vi "截取字符串.vi"(0 "T 1":T2, 1 "标刻内容 2":T1, 5 "T 2":T2, 9 "T 3":T2, 11 "T 4":T2, 12 "T 5":T2, 13 "T 6":T2) -> (4 "标刻内容":T1)   [LabVIEW 2021]
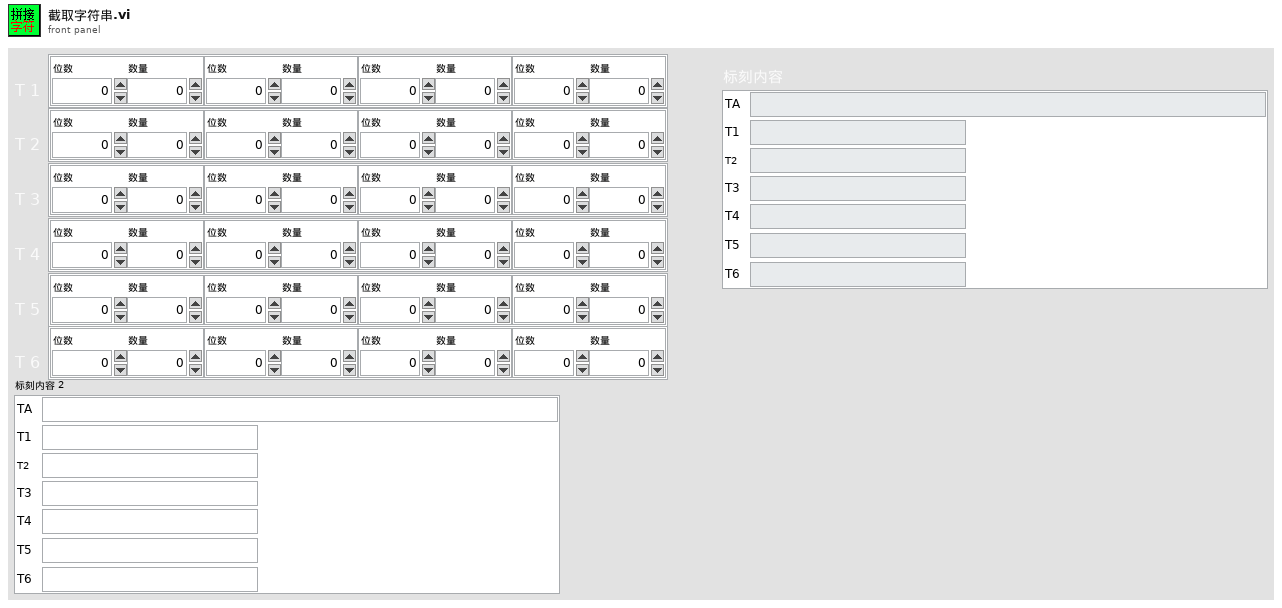
[diagram p1: front panel]
types:
  T1 = typedef "标刻内容.ctl" = cluster{"T1":string, "T2":string, "T3":string, "T4":string, "TA":string, "T5":string, "T6":string}
  T2 = typedef "T码提取设置.ctl" = cluster{"T1 1":cluster{"位数":dbl, "数量":dbl}, "T1 2":cluster{"位数":dbl, "数量":dbl}, "T1 3":cluster{"位数":dbl, "数量":dbl}, "T1 4":cluster{"位数":dbl, "数量":dbl}}
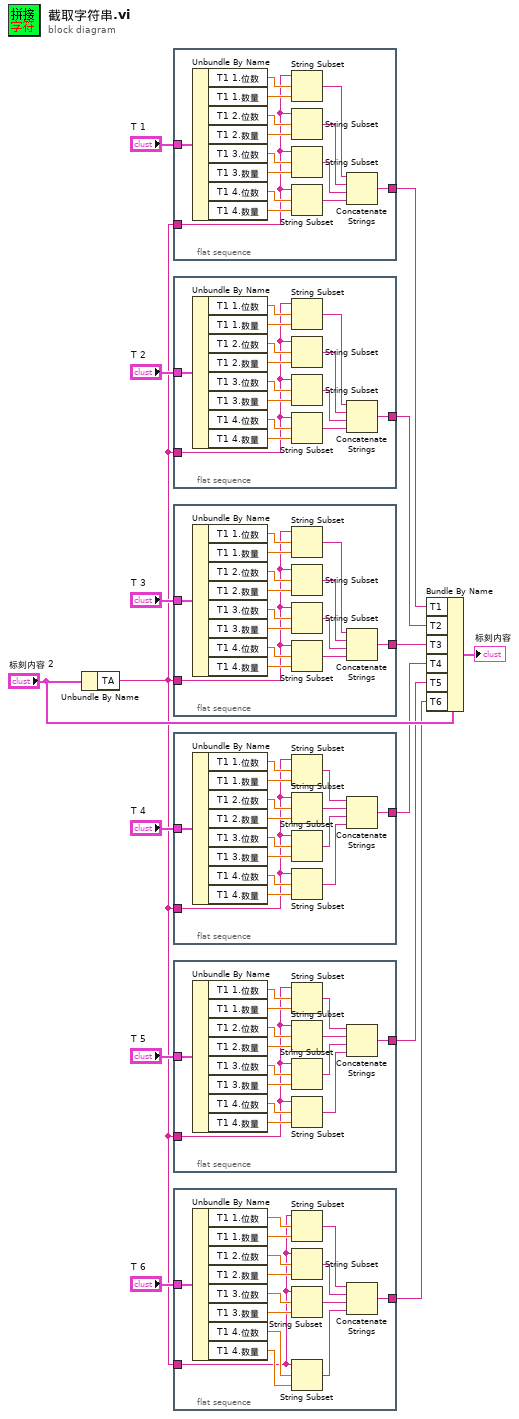
[diagram p0: block diagram]
diagram:
  n1 = Unbundle By Name("标刻内容 2") -> ("TA"=w6:string)
  n2 = flat-sequence {
    tunnel: "T 1" -> [w30]
    tunnel: w6 -> [w21]
    tunnel: [w16] -> w12
    frame #0 {
      n3 = Unbundle By Name(w30) -> ("T1 1.位数"=w29:dbl, "T1 1.数量"=w28:dbl, "T1 2.位数"=w27:dbl, "T1 2.数量"=w26:dbl, "T1 3.位数"=w25:dbl, "T1 3.数量"=w24:dbl, "T1 4.位数"=w23:dbl, "T1 4.数量"=w22:dbl)
      n4 = String Subset(string=w21, offset (0)=w29, length (rest)=w28) -> (substring=w20:string)
      n5 = String Subset(string=w21, offset (0)=w27, length (rest)=w26) -> (substring=w19:string)
      n6 = String Subset(string=w21, offset (0)=w25, length (rest)=w24) -> (substring=w18:string)
      n7 = String Subset(string=w21, offset (0)=w23, length (rest)=w22) -> (substring=w17:string)
      n8 = Concatenate Strings(w20, w19, w18, w17) -> (w16:string)
    }
  }
  n9 = flat-sequence {
    tunnel: "T 2" -> [w45]
    tunnel: [w32] -> w5
    tunnel: w6 -> [w31]
    frame #0 {
      n10 = Unbundle By Name(w45) -> ("T1 1.位数"=w44:dbl, "T1 1.数量"=w43:dbl, "T1 2.位数"=w42:dbl, "T1 2.数量"=w41:dbl, "T1 3.位数"=w40:dbl, "T1 3.数量"=w39:dbl, "T1 4.位数"=w38:dbl, "T1 4.数量"=w37:dbl)
      n11 = String Subset(string=w31, offset (0)=w44, length (rest)=w43) -> (substring=w36:string)
      n12 = String Subset(string=w31, offset (0)=w42, length (rest)=w41) -> (substring=w35:string)
      n13 = String Subset(string=w31, offset (0)=w40, length (rest)=w39) -> (substring=w34:string)
      n14 = String Subset(string=w31, offset (0)=w38, length (rest)=w37) -> (substring=w33:string)
      n15 = Concatenate Strings(w36, w35, w34, w33) -> (w32:string)
    }
  }
  n16 = flat-sequence {
    tunnel: "T 3" -> [w60]
    tunnel: w6 -> [w51]
    tunnel: [w46] -> w4
    frame #0 {
      n17 = Unbundle By Name(w60) -> ("T1 1.位数"=w59:dbl, "T1 1.数量"=w58:dbl, "T1 2.位数"=w57:dbl, "T1 2.数量"=w56:dbl, "T1 3.位数"=w55:dbl, "T1 3.数量"=w54:dbl, "T1 4.位数"=w53:dbl, "T1 4.数量"=w52:dbl)
      n18 = String Subset(string=w51, offset (0)=w59, length (rest)=w58) -> (substring=w50:string)
      n19 = String Subset(string=w51, offset (0)=w57, length (rest)=w56) -> (substring=w49:string)
      n20 = String Subset(string=w51, offset (0)=w55, length (rest)=w54) -> (substring=w48:string)
      n21 = String Subset(string=w51, offset (0)=w53, length (rest)=w52) -> (substring=w47:string)
      n22 = Concatenate Strings(w50, w49, w48, w47) -> (w46:string)
    }
  }
  n23 = flat-sequence {
    tunnel: "T 4" -> [w75]
    tunnel: w6 -> [w66]
    tunnel: [w61] -> w3
    frame #0 {
      n24 = Unbundle By Name(w75) -> ("T1 1.位数"=w74:dbl, "T1 1.数量"=w73:dbl, "T1 2.位数"=w72:dbl, "T1 2.数量"=w71:dbl, "T1 3.位数"=w70:dbl, "T1 3.数量"=w69:dbl, "T1 4.位数"=w68:dbl, "T1 4.数量"=w67:dbl)
      n25 = String Subset(string=w66, offset (0)=w74, length (rest)=w73) -> (substring=w65:string)
      n26 = String Subset(string=w66, offset (0)=w72, length (rest)=w71) -> (substring=w64:string)
      n27 = String Subset(string=w66, offset (0)=w70, length (rest)=w69) -> (substring=w63:string)
      n28 = String Subset(string=w66, offset (0)=w68, length (rest)=w67) -> (substring=w62:string)
      n29 = Concatenate Strings(w65, w64, w63, w62) -> (w61:string)
    }
  }
  n30 = flat-sequence {
    tunnel: "T 5" -> [w90]
    tunnel: w6 -> [w81]
    tunnel: [w76] -> w2
    frame #0 {
      n31 = Unbundle By Name(w90) -> ("T1 1.位数"=w89:dbl, "T1 1.数量"=w88:dbl, "T1 2.位数"=w87:dbl, "T1 2.数量"=w86:dbl, "T1 3.位数"=w85:dbl, "T1 3.数量"=w84:dbl, "T1 4.位数"=w83:dbl, "T1 4.数量"=w82:dbl)
      n32 = String Subset(string=w81, offset (0)=w89, length (rest)=w88) -> (substring=w80:string)
      n33 = String Subset(string=w81, offset (0)=w87, length (rest)=w86) -> (substring=w79:string)
      n34 = String Subset(string=w81, offset (0)=w85, length (rest)=w84) -> (substring=w78:string)
      n35 = String Subset(string=w81, offset (0)=w83, length (rest)=w82) -> (substring=w77:string)
      n36 = Concatenate Strings(w80, w79, w78, w77) -> (w76:string)
    }
  }
  n37 = flat-sequence {
    tunnel: "T 6" -> [w105]
    tunnel: w6 -> [w96]
    tunnel: [w91] -> w1
    frame #0 {
      n38 = Unbundle By Name(w105) -> ("T1 1.位数"=w104:dbl, "T1 1.数量"=w103:dbl, "T1 2.位数"=w102:dbl, "T1 2.数量"=w101:dbl, "T1 3.位数"=w100:dbl, "T1 3.数量"=w99:dbl, "T1 4.位数"=w98:dbl, "T1 4.数量"=w97:dbl)
      n39 = String Subset(string=w96, offset (0)=w104, length (rest)=w103) -> (substring=w95:string)
      n40 = String Subset(string=w96, offset (0)=w102, length (rest)=w101) -> (substring=w94:string)
      n41 = String Subset(string=w96, offset (0)=w100, length (rest)=w99) -> (substring=w93:string)
      n42 = String Subset(string=w96, offset (0)=w98, length (rest)=w97) -> (substring=w92:string)
      n43 = Concatenate Strings(w95, w94, w93, w92) -> (w91:string)
    }
  }
  n44 = Bundle By Name(cluster="标刻内容 2", "T1"=w12, "T2"=w5, "T3"=w4, "T4"=w3, "T5"=w2, "T6"=w1) -> (→"标刻内容":T1)
